vi "PicoScope6000aGetValuesOverlapped.vi"(5 "Segment Range":T1 {"toSegmentIndex" format="%.4p"; "fromSegmentIndex" format="%.4p"}, 7 "Buffer and Transfer Settings":T2 {"Down-Sample Mode" items=["None", "Aggregate", "Decimate", "Average"]; "Down Sample Ratio" step=1; "Samples" format="%_6p"}, 8 "error in (no error)":errorcluster, 11 "handle in":i16) -> (0 "error out":errorcluster, 3 "handle out":i16, 4 "overflow":i16 format="%010b", 6 "noOfSamples":u64)   [LabVIEW 2009]
doc: "Calls ps6000aGetValues"
uses:
  ps6000a.dll
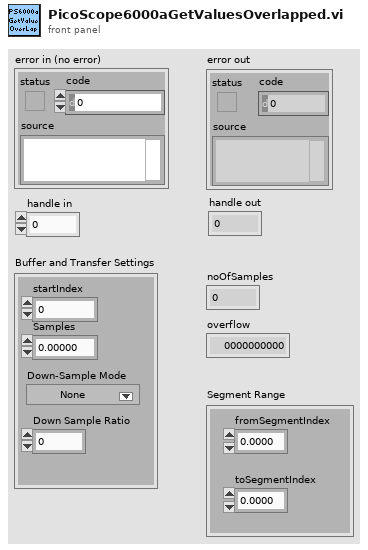
[diagram p1: front panel]
types:
  T1 = cluster{"fromSegmentIndex":u64, "toSegmentIndex":u64}
  T2 = cluster{"startIndex":u64, "Samples":u64, "Down Sample Ratio":u64, "Down-Sample Mode":u32}
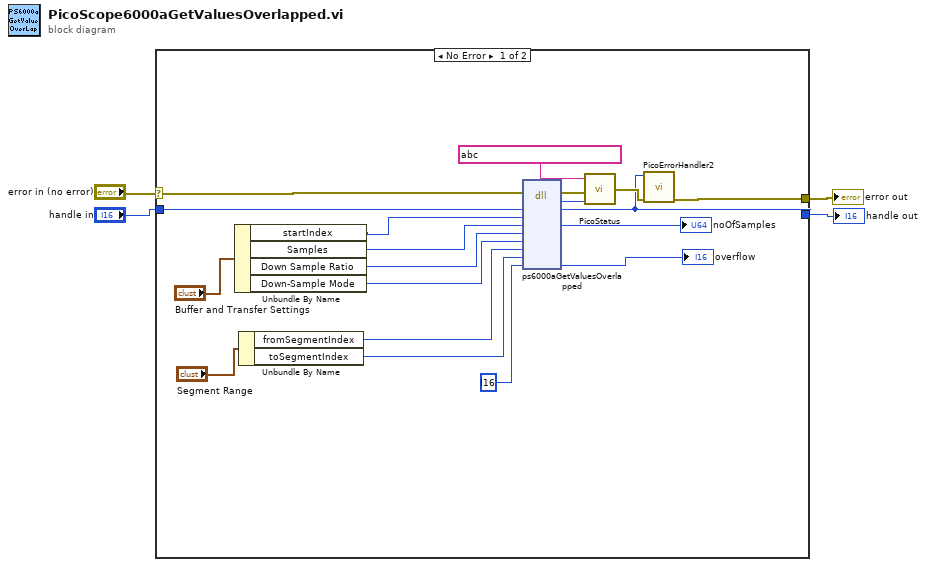
[diagram p0: block diagram]
diagram:
  n1 = case shown="No Error" "error in (no error)" {
    selector: "error in (no error)" -> [w13 w24]
    tunnel: "handle in" -> [w12 w25]
    tunnel: [w10 w25] -> w4
    tunnel: [w11 w24] -> w3
    frame #0 {
      n2 = Unbundle By Name("Buffer and Transfer Settings") -> ("startIndex"=w14:u64, "Samples"=w23:u64, "Down Sample Ratio"=w20:u64, "Down-Sample Mode"=w21:u32)
      n3 = Unbundle By Name("Segment Range") -> ("fromSegmentIndex"=w7:u64, "toSegmentIndex"=w6:u64)
      n4 = dll-call lib="ps6000a.dll" fn="ps6000aGetValuesOverlapped" ("ps3000.dll:_ps3000_open_unit@0")(error in=w13, "handle"=w12, "startIndex"=w14, "noOfSamples"=w23, "downSampleRatio"=w20, "downSampleRatioMode"=w21, "fromSegmentIndex"=w7, "toSegmentIndex"=w6, "overflow"=i16 ?) -> (error out=w19:errorcluster, "PICO_STATUS"=w18:u32, "handle"=w10:i16, "noOfSamples"=→"noOfSamples":u64, "overflow"=→"overflow":i16)  [unwired: 7 in, 1 out]
      n5 = call "PicoStatus.vi"("PICO STATUS"=w18, "error in"=w19, "source"=string ?) -> ("error out"=w22:errorcluster)
      n6 = call "PicoErrorHandler2.vi"("error in (no error)"=w22, "handle In"=w10) -> ("error out"=w11:errorcluster)  [unwired: 9 in]
    }
    frame #1 {
    }
  }
  "error out" <- w3
  "handle out" <- w4
